vi "Parse Bitfile for EST IP.vi"(8 "error in (no error)":errorcluster, 9 "RIO device address":string, 10 "bitfile path":path, 11 "Item Ref in":T1 format="%.0x") -> (0 "error out":errorcluster, 1 "APUs":string[](array[string]), 2 "version":string, 3 "Item Ref out":T1 format="%.0x")   [LabVIEW 2020, in "Engine Simulation Toolkit System Explorer.lvlib"]
uses:
  Engine Simulation Toolkit System Explorer.lvlib
  <vilib>/NI VeriStand/Custom Device API/Custom Device Item Ref.ctl
  Shared/Properties.vi
  Shared/Constants and GUIDs.vi
  <vilib>/NI VeriStand/Custom Device API/Set Item Property (String).vi
  <vilib>/NI VeriStand/Custom Device API/Custom Device API.lvlib
  Shared/Engine Simulation Toolkit Shared.lvlib
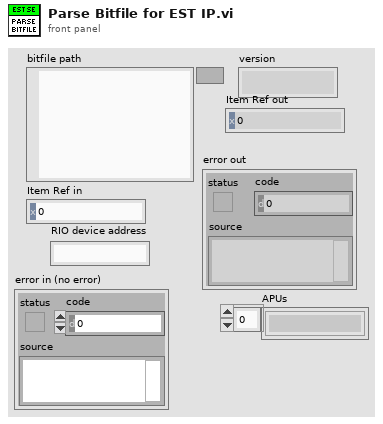
[diagram p1: front panel]
types:
  T1 = typedef "Custom Device API.lvlib/Custom Device Item Ref.ctl" = u64
  T2 = typedef "Engine Simulation Toolkit Shared.lvlib/Bitfile EST Version.ctl" = enum16{"1.0", "1.1", "1.2", "1.3", "1.4"}
  T3 = typedef "Engine Simulation Toolkit System Explorer.lvlib/String Array Property.ctl" = cluster{"Property Name":string, "Property Value":string[]}
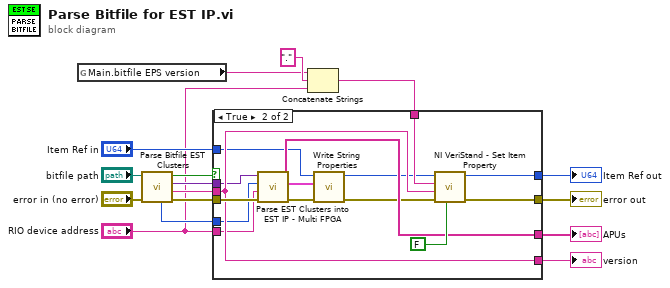
[diagram p0: block diagram]
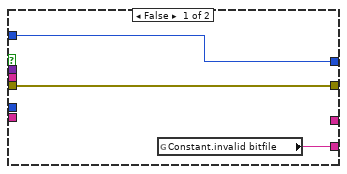
[diagram p2: hidden frame]
diagram:
  n1 = global read "Properties.vi" "Main.bitfile EPS version"() -> (w3:string)
  n2 = call "Parse Bitfile EST Clusters.vi"("error in (no error)"="error in (no error)", "bitfile path"="bitfile path") -> ("error out"=w16:errorcluster, "version"=w12:string, "EPS IP LUT"=w14:variant, "valid bitfile"=w7:bool, "EST version enum"=w5:T2)  [unwired: 5 in]
  n3 = Concatenate Strings(w3, "." ("string"), "RIO device address") -> (w1:string)
  n4 = case shown="True" w7 {
    tunnel: w16 -> [w19 w34]
    tunnel: w14 -> [_ w27]
    tunnel: "Item Ref in" -> [w18 w22]
    tunnel: w1 -> [_ w33]
    tunnel: w12 -> [_ w30]
    tunnel: [w19 w32] -> w10
    tunnel: [w18 w31] -> w8
    tunnel: [_ w28] -> w9
    tunnel: [w17 w30] -> w6
    tunnel: w5 -> [_ w26]
    tunnel: "RIO device address" -> [_ w20]
    frame False {
      n5 = global read "Constants and GUIDs.vi" "Constant.invalid bitfile"() -> (w17:string)
    }
    frame True {
      n6 = call "Parse EST Clusters into EST IP - Multi FPGA.vi"("error in (no error)"=w34, "RIO device address"=w20, "EST version enum"=w26, "EPS IP LUT"=w27) -> ("error out"=w24:errorcluster, "Properties"=w25:T3[], "APUs"=w28:string[])  [unwired: 5 in]
      n7 = call "Write String Properties.vi"("error in (no error)"=w24, "String Array Properties"=w25, "Item Ref in in"=w22) -> ("error out"=w23:errorcluster, "Item Ref out"=w21:T1)  [unwired: 7 in]
      n8 = call-poly <vilib>:"NI VeriStand - Set Item Property.vi"("Binary String (T)"=FALSE, "error in (no error)"=w23, "Value"=w30, "Property Name"=w33, "Item Ref in"=w21) -> ("error out"=w32:errorcluster, "Item Ref out"=w31:T1)  [unwired: 4 in, 1 out]
    }
  }
  "version" <- w6
  "error out" <- w10
  "Item Ref out" <- w8
  "APUs" <- w9
